vi "to_string.vi"(8 "error in (no error)":errorcluster, 11 "toml in":refnum<class "toml.lvclass">) -> (0 "error out":errorcluster, 2 "toml_string":string)   [LabVIEW 2020, in "toml.lvclass"]
uses:
  toml.lvclass
  toml.lvclass/toml.ctl
  Doc/Doc.lvclass
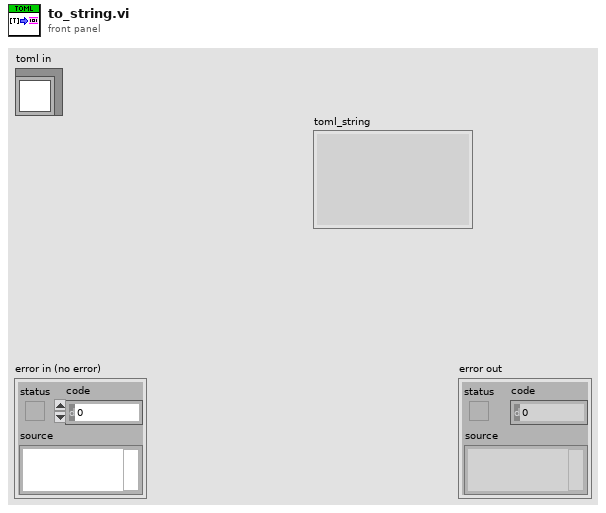
[diagram p1: front panel]
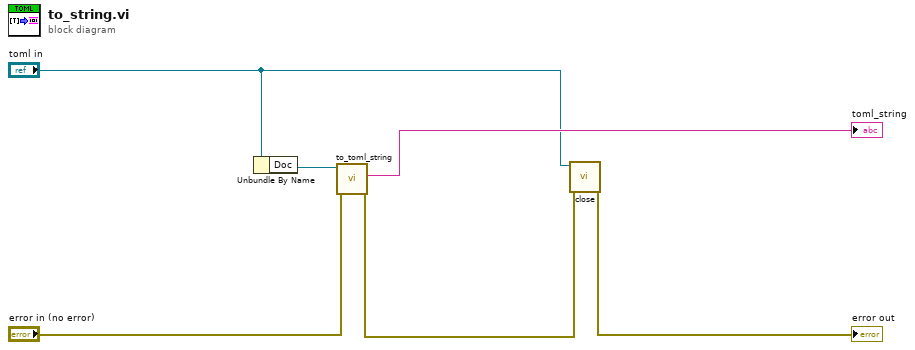
[diagram p0: block diagram]
diagram:
  n1 = Unbundle By Name("toml in") -> ("Doc"=w2:refnum<class "Doc.lvclass">)
  n2 = call "to_toml_string.vi"("error in (no error)"="error in (no error)", "Doc in"=w2) -> ("error out"=w3:errorcluster, "toml_string"=→"toml_string":string)  [unwired: 7 in, 1 out]
  n3 = call "close.vi"("error in (no error)"=w3, "toml in"="toml in") -> ("error out"=→"error out":errorcluster)  [unwired: 9 in]
